vi "GDSString_FindWord.vi"(0 "Text":string, 1 "StringStartOffset(Default=-1 => 0 for Forward, StrLenght for Backwards)":i32=-1, 2 "PatternMatchingDelimiter(\\s\\t\\r\\n)":string="\\s\\t\\r\\n", 3 "Search Backwards":bool, 4 "AllowedWords(PatternMatching)":string[](array[string]), 5 "error in (no error)":errorcluster, 6 "GetNext-X_Words(1,-1=All)":i32=1, 7 "ExactWord":bool=TRUE, 8 "IgnoreMatchesWithinThesePositions":i32[][](array[numeric])) -> (14 "NextWord":string, 15 "IndexAfterMatch(Or before when searching Backwards)":i32=1, 16 "NextWords":string[](array[string]), 17 "IndexAfterMatches(Or before when searching Backwards)":i32[](array[numeric]), 18 "IndexAfterLastMatch(Or before when searching Backwards)":i32=1, 19 "error out":errorcluster)   [LabVIEW 2020]
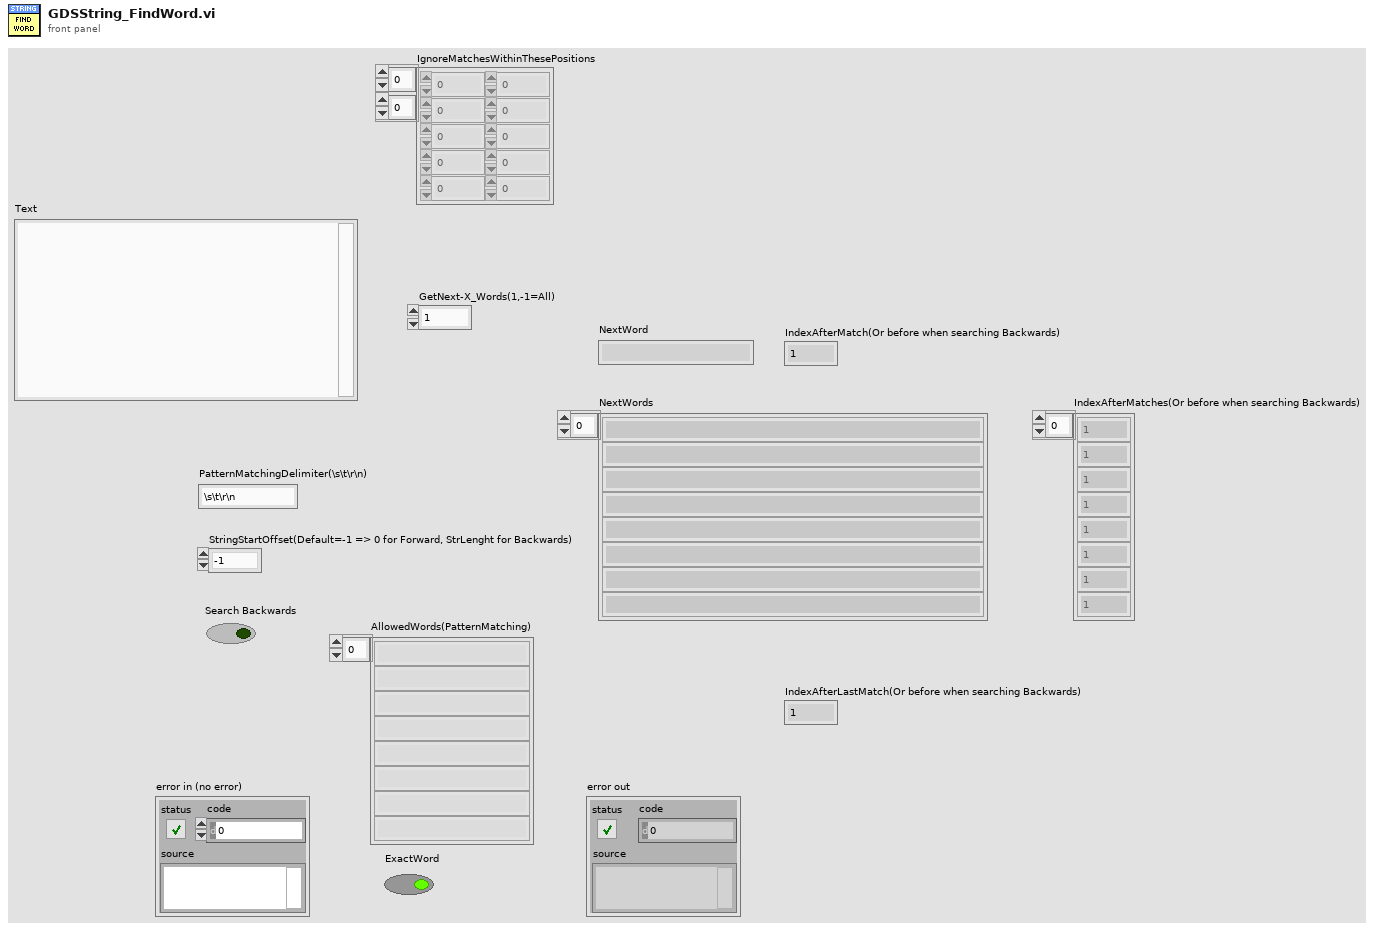
[diagram p1: front panel]
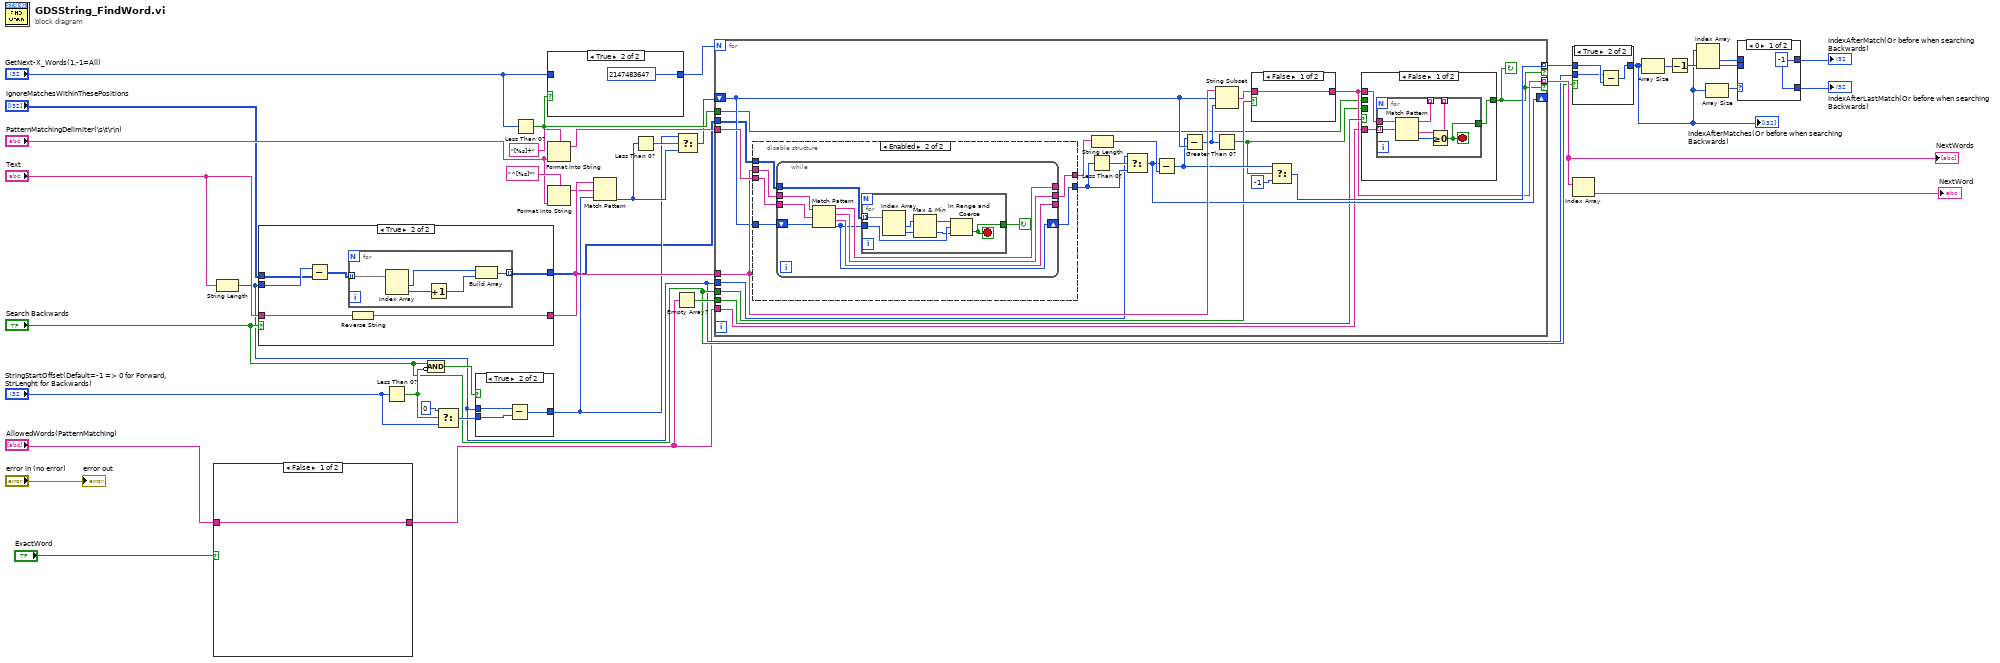
[diagram p0: block diagram]
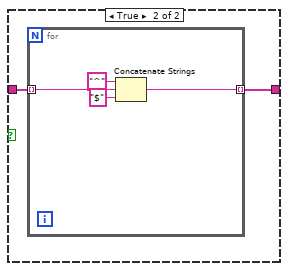
[diagram p3: hidden frame]
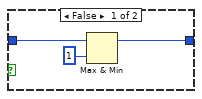
[diagram p5: hidden frame]
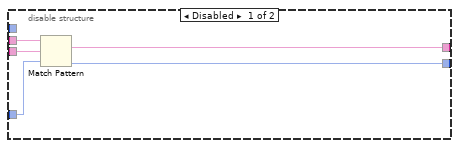
[diagram p6: hidden frame]
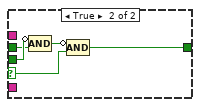
[diagram p7: hidden frame]
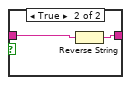
[diagram p8: hidden frame]
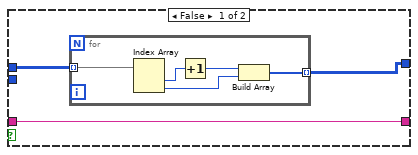
[diagram p10: hidden frame]
diagram:
  n1 = case shown="False" "ExactWord" {
    tunnel: "AllowedWords(PatternMatching)" -> [w40 w42]
    tunnel: [w40 w41] -> w8
    frame False {
    }
    frame True {
      n2 = for {
        tunnel: w42 -> [w46] mode=indexing
        tunnel: [w45] -> w41 mode=indexing
        n3 = Concatenate Strings("^" ("string"), w46, "$" ("string")) -> (w45:string)
      }
    }
  }
  n4 = String Length(string="Text") -> (length=w11:i32)
  n5 = case shown="True" "Search Backwards" {
    tunnel: "Text" -> [w49 w60]
    tunnel: [w49 w59] -> w33
    tunnel: "IgnoreMatchesWithinThesePositions" -> [w48 w57]
    tunnel: [w47 w55] -> w13
    tunnel: w11 -> [_ w58]
    frame False {
      n6 = for {
        tunnel: w48 -> [w54] mode=indexing
        tunnel: [w52] -> w47 mode=indexing
        n7 = Index Array(array=w54) -> (element #1=w51:i32, element #2=w53:i32)  [unwired: 2 in]
        n8 = Increment(x=w51) -> (x+1=w50:i32)
        n9 = Build Array(w50, w53) -> (w52:i32[])
      }
    }
    frame True {
      n10 = Subtract(x=w58, y=w57) -> (x-y=w56:i32[][])
      n11 = for {
        tunnel: w56 -> [w65] mode=indexing
        tunnel: [w63] -> w55 mode=indexing
        n12 = Index Array(array=w65) -> (element #1=w64:i32, element #2=w62:i32)  [unwired: 2 in]
        n13 = Increment(x=w62) -> (x+1=w61:i32)
        n14 = Build Array(w64, w61) -> (w63:i32[])
      }
      n15 = Reverse String(1:w60) -> (0:w59:string)
    }
  }
  n16 = Less Than 0?(x="StringStartOffset(Default=-1 => 0 for Forward, StrLenght for Backwards)") -> (x < 0?=w16:bool)
  n17 = Compound Arithmetic op=AND("Search Backwards", invert w16) -> (w14:bool)
  n18 = Select(t=0, s=w16, f="StringStartOffset(Default=-1 => 0 for Forward, StrLenght for Backwards)") -> (s? t:f=w18:i32)
  n19 = case shown="True" w14 {
    tunnel: w18 -> [w66 w68]
    tunnel: [w66 w67] -> w17
    tunnel: w11 -> [_ w69]
    frame False {
    }
    frame True {
      n20 = Subtract(x=w69, y=w68) -> (x-y=w67:i32)
    }
  }
  n21 = Less Than 0?(x="GetNext-X_Words(1,-1=All)") -> (x < 0?=w22:bool)
  n22 = case shown="True" w22 {
    tunnel: [w71 2147483647] -> w34
    tunnel: "GetNext-X_Words(1,-1=All)" -> [w70 _]
    frame False {
      n23 = Max & Min(x=w70, y=1) -> (max(x,y)=w71:i32)  [unwired: 1 out]
    }
    frame True {
    }
  }
  n24 = Format Into String(format string="[%s]+", "PatternMatchingDelimiter(\\s\\t\\r\\n)") -> (resulting string=w37:string)  [unwired: 2 in, 1 out]
  n25 = Format Into String(format string="^[%s]*", "PatternMatchingDelimiter(\\s\\t\\r\\n)") -> (resulting string=w30:string)  [unwired: 2 in, 1 out]
  n26 = Match Pattern(string=w33, regular expression=w30, offset (0)=w17) -> (offset past match=w27:i32)  [unwired: 3 out]
  n27 = Less Than 0?(x=w27) -> (x < 0?=w28:bool)
  n28 = Empty Array?(array=w8) -> (empty?=w24:bool)
  n29 = Select(t=w17, s=w28, f=w27) -> (s? t:f=w19:i32)
  n30 = for {
    N: w34 -> [_]
    tunnel: w33 -> [w92]
    tunnel: w37 -> [w95]
    tunnel: [w83] -> w29 mode=indexing if=w77
    shift-right: [w87] -> _
    shift-left: w19 -> [w88]
    tunnel: w11 -> [w89]
    tunnel: [w79] -> w25 mode=indexing if=w77
    tunnel: "Search Backwards" -> [w82]
    tunnel: w24 -> [w80]
    tunnel: w8 -> [w78]
    tunnel: w22 -> [w75]
    tunnel: w13 -> [w74]
    stop <- w77 continue-if-true
    n31 = disable-structure shown="Enabled" {
      disable-tunnel: w95 -> [w100 w105]
      disable-tunnel: [w99 w102] -> w94
      disable-tunnel: w92 -> [w98 w106]
      disable-tunnel: [w97 w103] -> w90
      disable-tunnel: w88 -> [w96 w104]
      disable-tunnel: w74 -> [_ w101]
      frame Disabled {
        n32 = Match Pattern(string=w98, regular expression=w100, offset (0)=w96) -> (match substring=w99:string, offset past match=w97:i32)  [unwired: 2 out]
      }
      frame Enabled {
        n33 = while {
          tunnel: w106 -> [w115]
          tunnel: [w114] -> _
          tunnel: [w113] -> _
          tunnel: w105 -> [w112]
          tunnel: [w110] -> w102
          shift-right: [w109] -> w103
          shift-left: w104 -> [w111]
          tunnel: w101 -> [w108]
          stop <- w107 continue-if-true
          n34 = Match Pattern(string=w115, regular expression=w112, offset (0)=w111) -> (before substring=w113:string, match substring=w110:string, after substring=w114:string, offset past match=w109:i32)
          n35 = for {
            tunnel: w108 -> [w121] mode=indexing
            tunnel: w109 -> [w122]
            tunnel: [w120] -> w107
            stop <- w120 stop-if-true
            n36 = Index Array(array=w121) -> (element #1=w117:i32, element #2=w116:i32)  [unwired: 2 in]
            n37 = Max & Min(x=w117, y=w116) -> (max(x,y)=w119:i32, min(x,y)=w118:i32)
            n38 = In Range and Coerce(upper limit=w119, x=w122, lower limit=w118) -> (In Range?=w120:bool)  [unwired: 1 out]
          }
        }
      }
    }
    n39 = Less Than 0?(x=w90) -> (x < 0?=w91:bool)
    n40 = String Length(string=w94) -> (length=w93:i32)
    n41 = Select(t=w89, s=w91, f=w90) -> (s? t:f=w87:i32)
    n42 = Subtract(x=w87, y=w93) -> (x-y=w85:i32)
    n43 = Subtract(x=w85, y=w88) -> (x-y=w86:i32)
    n44 = String Subset(string=w92, offset (0)=w88, length (rest)=w86) -> (substring=w81:string)
    n45 = Greater Than 0?(x=w86) -> (x > 0?=w76:bool)
    n46 = case shown="False" w82 {
      tunnel: w81 -> [w137 w139]
      tunnel: [w137 w138] -> w79
      frame False {
      }
      frame True {
        n47 = Reverse String(1:w139) -> (0:w138:string)
      }
    }
    n48 = Select(t=w85, s=w76, f=-1) -> (s? t:f=w83:i32)
    n49 = case shown="False" w80 {
      selector: w80 -> [_ w136]
      tunnel: [w123 w135] -> w77
      tunnel: w79 -> [w125 _]
      tunnel: w78 -> [w124 _]
      tunnel: w76 -> [_ w134]
      tunnel: w75 -> [_ w133]
      frame False {
        n50 = for {
          tunnel: w125 -> [w131]
          tunnel: w124 -> [w130] mode=indexing
          tunnel: [w128] -> w123
          tunnel: [w127] -> _ mode=indexing
          tunnel: [w126] -> _ mode=indexing
          stop <- w128 stop-if-true
          n51 = Match Pattern(string=w131, regular expression=w130) -> (before substring=w127:string, after substring=w126:string, offset past match=w129:i32)  [unwired: 1 in, 1 out]
          n52 = Greater Or Equal To 0?(x=w129) -> (x >= 0?=w128:bool)
        }
      }
      frame True {
        n53 = Compound Arithmetic op=AND(invert w134, w133) -> (w132:bool)
        n54 = Compound Arithmetic op=AND(invert w132, w136) -> (w135:bool)
      }
    }
  }
  "NextWords" <- w25
  n55 = case shown="True" "Search Backwards" {
    tunnel: w29 -> [w140 w143]
    tunnel: [w140 w141] -> w6
    tunnel: w11 -> [_ w142]
    frame False {
    }
    frame True {
      n56 = Subtract(x=w142, y=w143) -> (x-y=w141:i32[])
    }
  }
  "IndexAfterMatches(Or before when searching Backwards)" <- w6
  n57 = Index Array(array=w25) -> (element=→"NextWord":string)  [unwired: 1 in]
  n58 = Array Size(array=w6) -> (size(s)=w21:i32)
  n59 = Decrement(x=w21) -> (x-1=w20:i32)
  n60 = Index Array(array=w6, index #2=w20) -> (element #1=w4:i32, element #2=w3:i32)  [unwired: 1 in]
  n61 = Array Size(array=w6) -> (size(s)=w5:i32)
  n62 = case shown="0" w5 {
    tunnel: w4 -> [_ w145]
    tunnel: w3 -> [_ w146]
    tunnel: [w144 w146] -> w2
    tunnel: [w144 w145] -> w1
    frame 0 {
      w144 = -1 ("f")
    }
    frame Default {
    }
  }
  "IndexAfterMatch(Or before when searching Backwards)" <- w1
  "IndexAfterLastMatch(Or before when searching Backwards)" <- w2
  "error out" <- "error in (no error)"
